vi "wiringPiI2CSetSlaveID.vi"(8 "error in (no error)":errorcluster, 10 "Slave Id":u8, 11 "devID":T1) -> (0 "error out":errorcluster, 2 "return":i32)   [LabVIEW 2020, in "wiringPi.lvlib"]
doc: "<b>_______________________________________________________________</b>\n** Author: Juan José Villacorta\n** LabVIEW wrapper for C library <b> wiringPi </b>,\n** https://github.com/WiringPi/WiringPi\n<b>_______________________________________________________________</b>\n\n/*\n * wiringPiI2CReadReg8: wiringPiI2CReadReg16:\n * Read a block of data from the device\n *********************************************************************************\n */"
uses:
  wiringPi.lvlib
  Type Defs/I2C Device.ctl
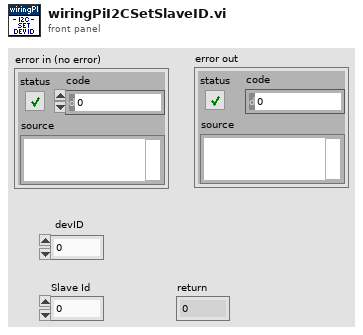
[diagram p1: front panel]
types:
  T1 = typedef "wiringPi.lvlib/I2C Device.ctl" = i32
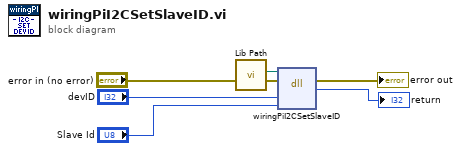
[diagram p0: block diagram]
diagram:
  n1 = call "Lib Path.vi"() -> ("path out"=w4:path)  [unwired: 11 in]
  n2 = dll-call lib="libLVwiringPI.so" fn="wiringPiI2CSetSlaveID"(path in=w4, error in="error in (no error)", "fd"="devID", "devId"="Slave Id") -> (error out=→"error out":errorcluster, "return type"=→"return":i32)  [unwired: 3 in, 1 out]
